vi "Post-Build Action.vi"(4 "measurement plugin service":refnum<class "Measurement Plugin Service.lvclass">, 5 "files generated by build":path[](array[path]), 6 "top level/always included VIs":path[](array[path]), 7 "destination path":path, 8 "error in":errorcluster, 9 "target name":string, 10 "build specification name":string, 11 "project path":path) -> (0 "error out":errorcluster)   [LabVIEW 2021, in "NI Measurement Plug-In SDK.lvlib"]
uses:
  NI Measurement Plug-In SDK.lvlib
  Measurement Plugin Service/Measurement Plugin Service.lvclass
  <vilib>/Utility/config.llb/Write Key (String).vi
  <vilib>/Utility/config.llb/NI_LVConfig.lvlib
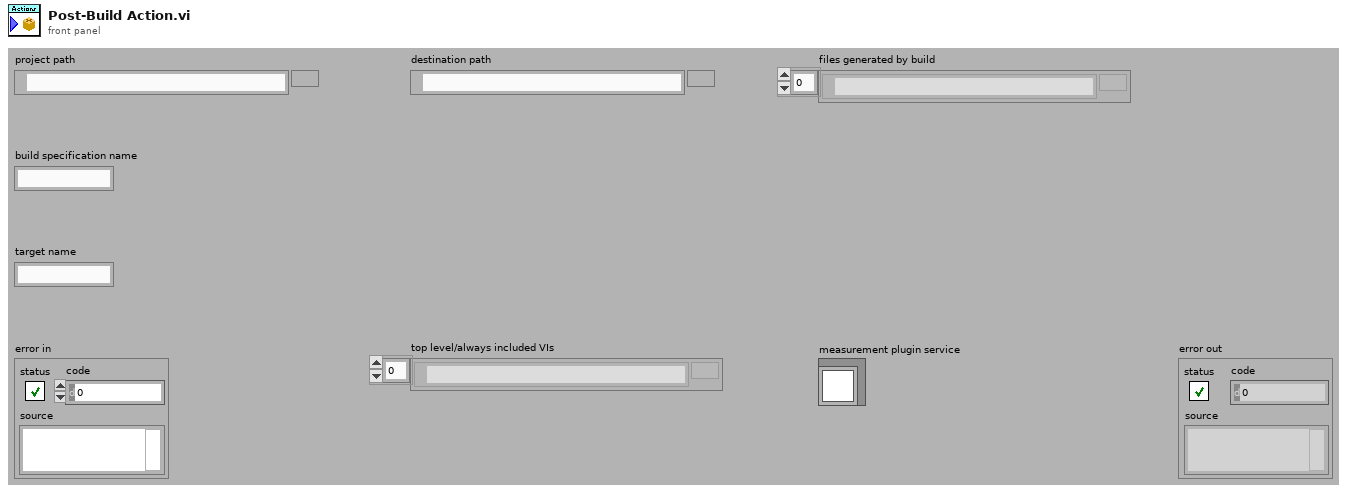
[diagram p1: front panel]
types:
  T1 = cluster{"target name":string, "top level/always included VIs":path[], "project path":path, "destination path":path, "build specification name":string, "files generated by build":path[]}
  T2 = typedef "NI Measurement Plug-In SDK.lvlib/User Interface Details.ctl" = cluster{"file url":string}
  T3 = typedef "NI Measurement Plug-In SDK.lvlib/Service Descriptor.ctl" = cluster{"measurement details":T4, "description URL":string, "service class":string, "measurement annotations":T5[]}
  T4 = typedef "NI Measurement Plug-In SDK.lvlib/Measurement Details.ctl" = cluster{"display name":string, "version":string}
  T5 = typedef "NI Measurement Plug-In SDK.lvlib/Measurement Annotation.ctl" = cluster{"key":string, "value":string}
  T6 = typedef "NI_LVConfig.lvlib/Config Data RefNum.ctl" = refnum<k1>
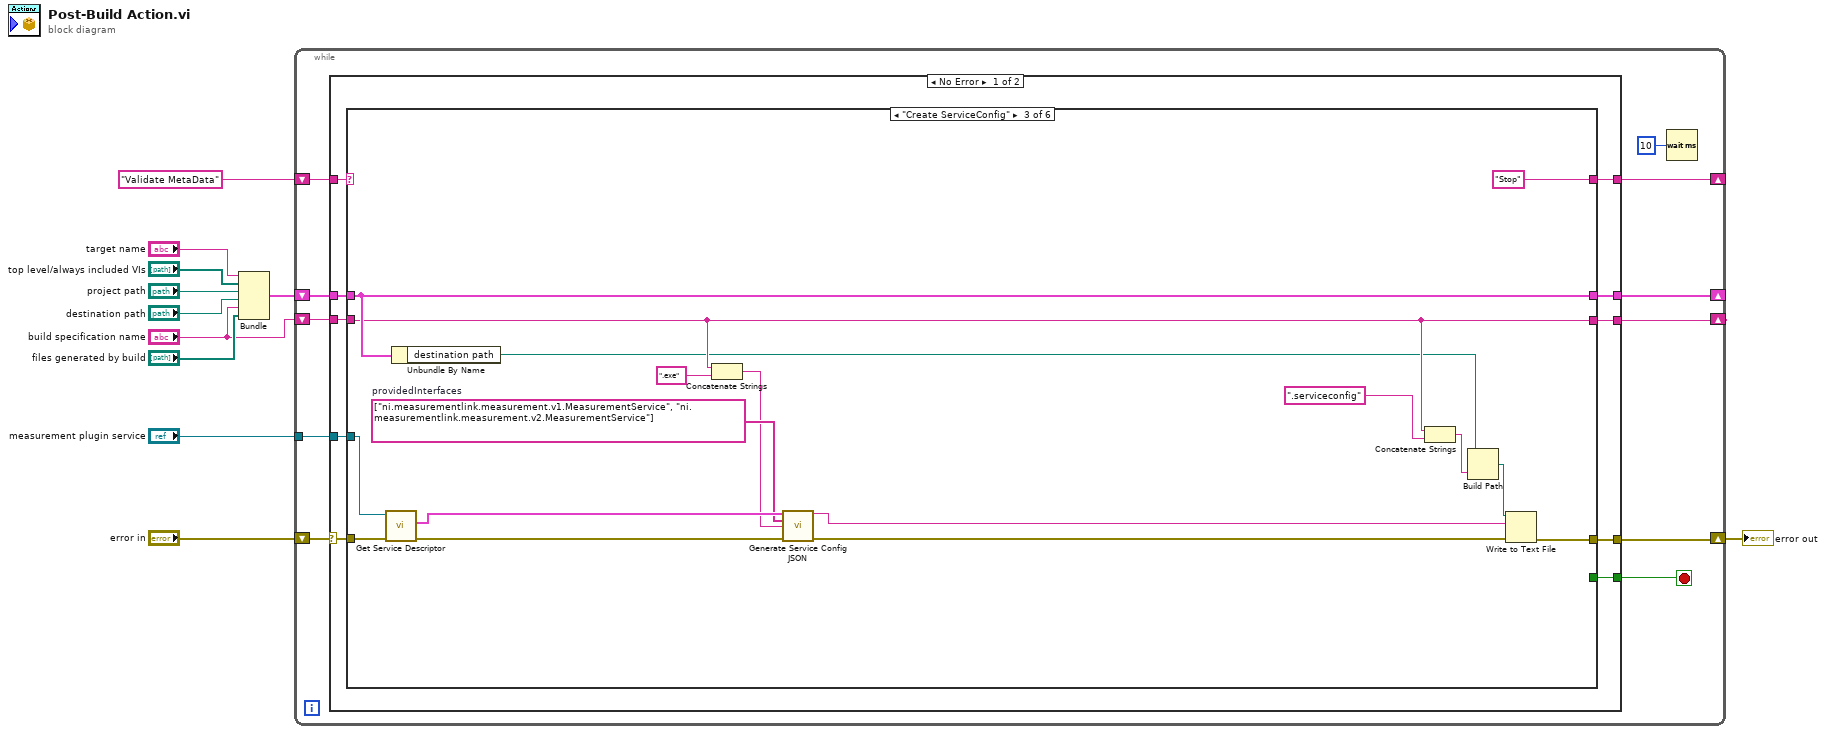
[diagram p0: block diagram]
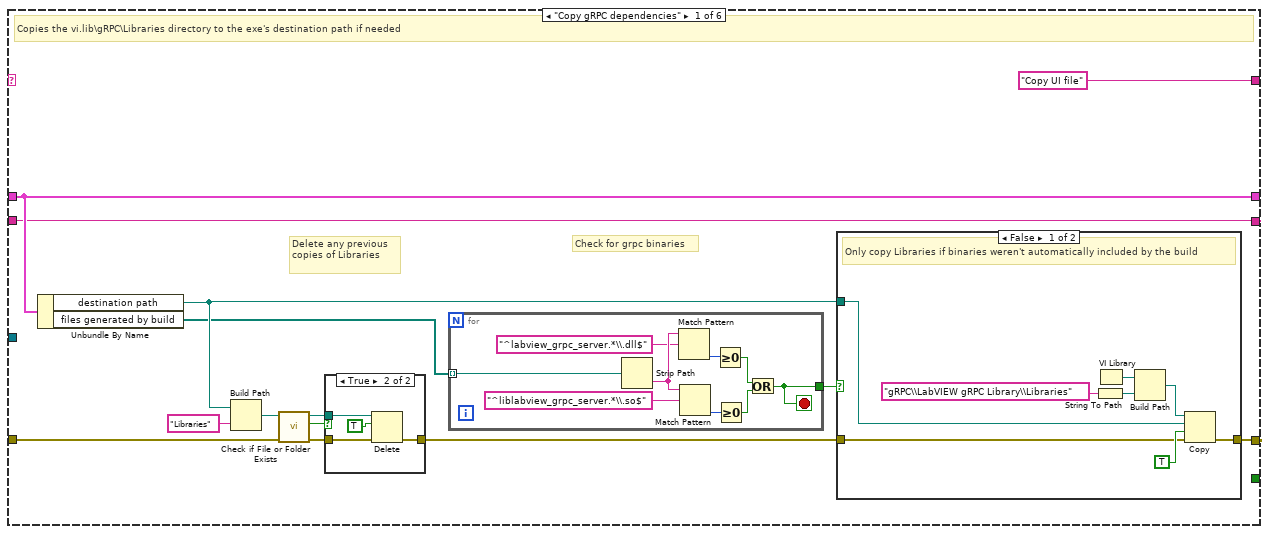
[diagram p2: hidden frame]
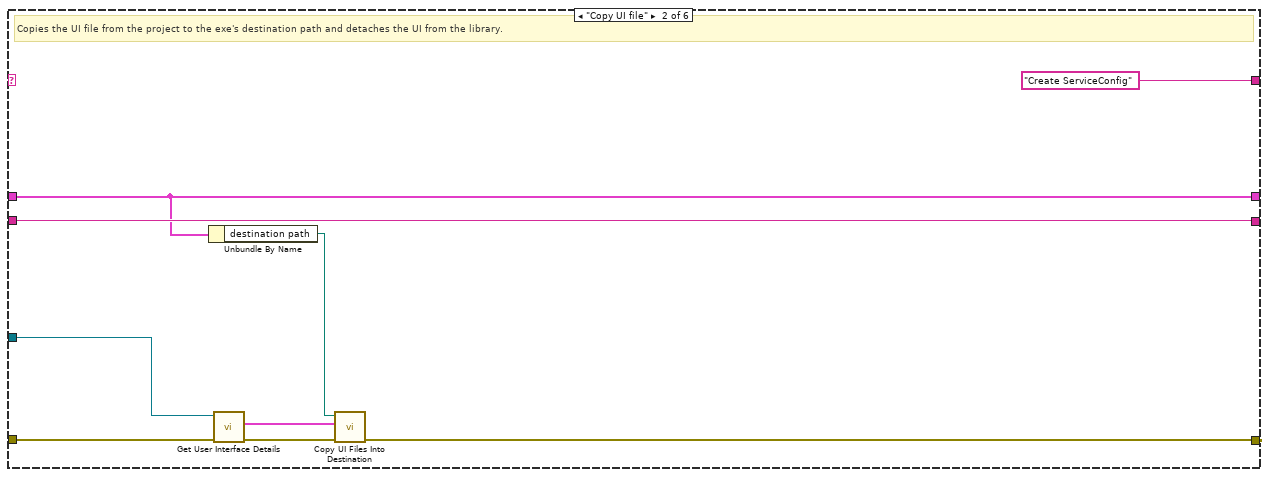
[diagram p5: hidden frame]
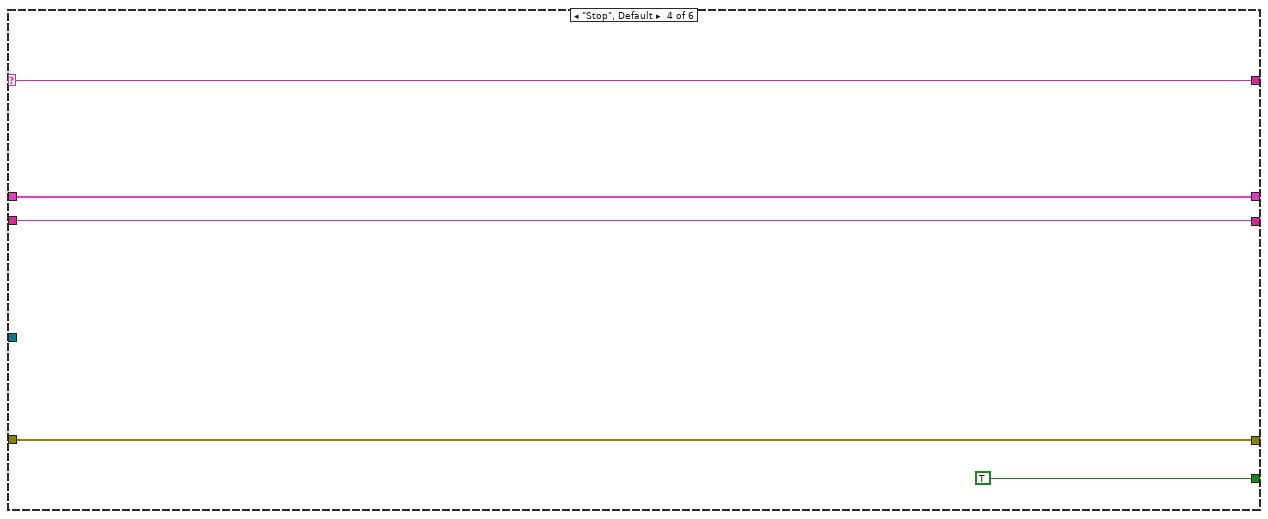
[diagram p6: hidden frame]
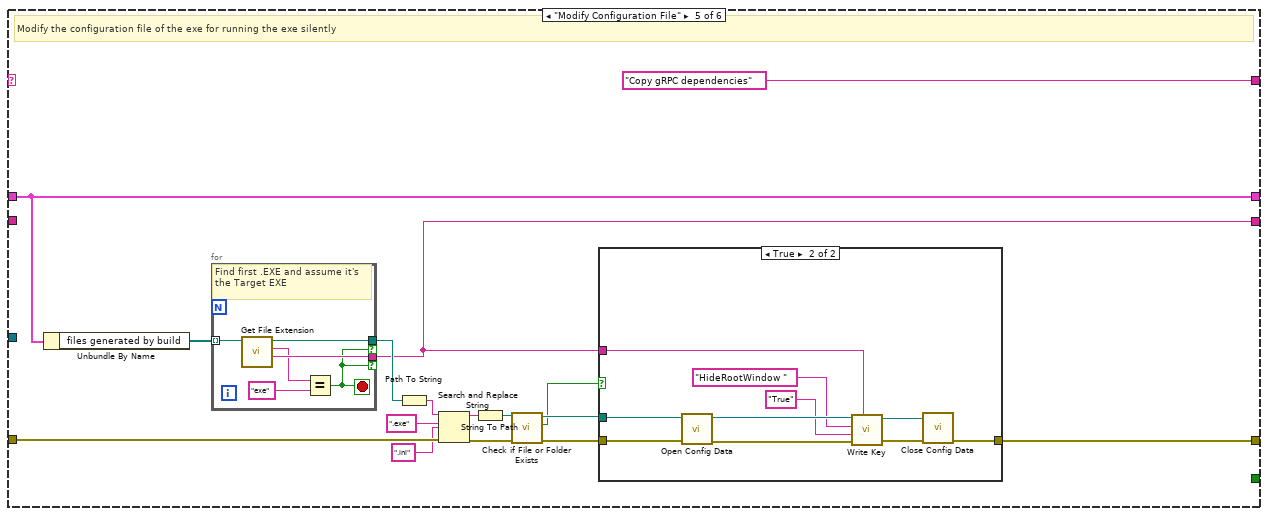
[diagram p7: hidden frame]
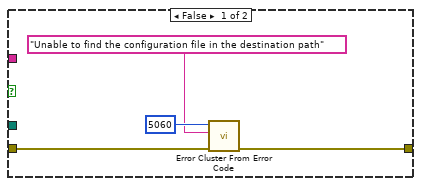
[diagram p8: hidden frame]
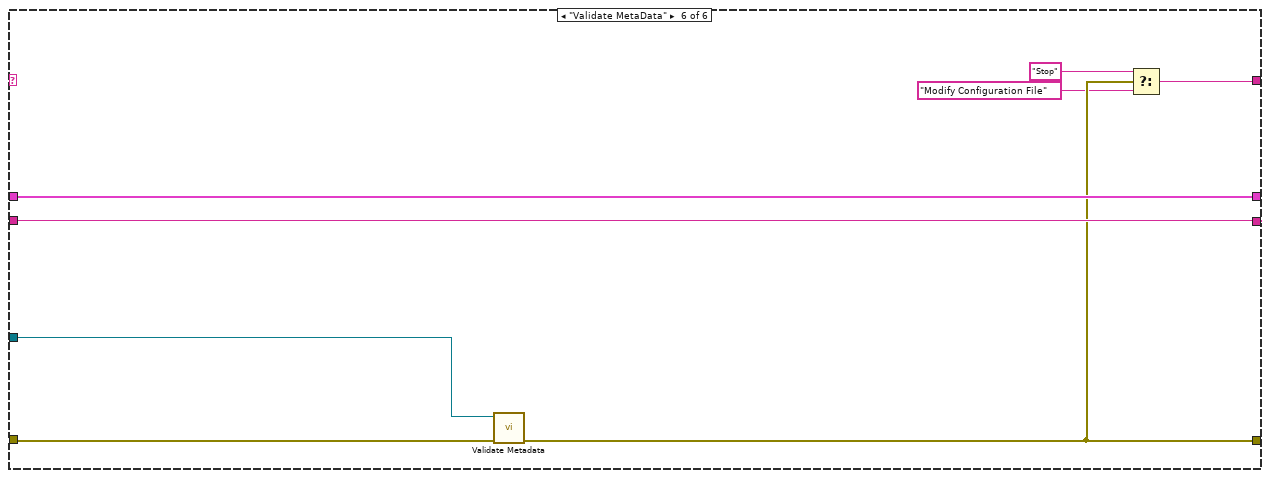
[diagram p9: hidden frame]
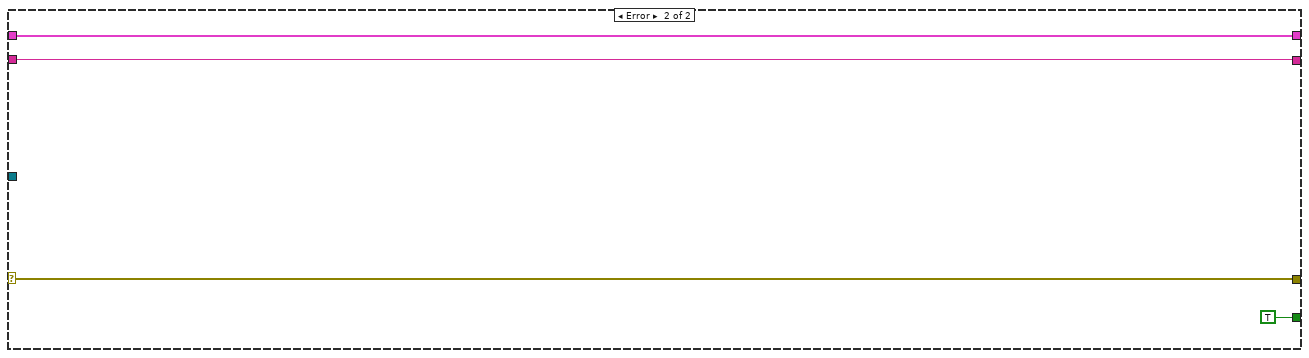
[diagram p10: hidden frame]
diagram:
  n1 = Bundle("target name"="target name", "top level/always included VIs"="top level/always included VIs", "project path"="project path", "destination path"="destination path", "build specification name"="build specification name", "files generated by build"="files generated by build") -> (w5:T1)  [unwired: 1 in]
  n2 = while {
    shift-right: [w19] -> _
    shift-left: w5 -> [w20]
    shift-right: [w18] -> w3
    shift-left: "error in" -> [w15]
    shift-right: [w17] -> _
    shift-left: "Validate MetaData" -> [w21]
    shift-right: [w14] -> _
    shift-left: "build specification name" -> [w13]
    tunnel: "measurement plugin service" -> [w12]
    stop <- w16 stop-if-true
    n3 = case shown="No Error" w15 {
      selector: w15 -> [w26 w147]
      tunnel: w21 -> [w32 _]
      tunnel: w20 -> [w31 w148]
      tunnel: [w30 w148] -> w19
      tunnel: [w29 w147] -> w18
      tunnel: [w28 _] -> w17
      tunnel: [w27 TRUE] -> w16
      tunnel: [w25 w145] -> w14
      tunnel: w13 -> [w24 w145]
      tunnel: w12 -> [w23 _]
      frame No Error {
        n4 = case shown="\"Create ServiceConfig\"" w32 {
          selector: w32 -> [_ _ _ w98 _ _]
          tunnel: w31 -> [w44 w75 w95 w100 w112 w144]
          tunnel: [w44 w75 w95 w100 w112 w144] -> w30
          tunnel: w26 -> [w36 w73 w85 w97 w110 w142]
          tunnel: [w46 w74 w88 w97 w116 w140] -> w29
          tunnel: ["Copy UI file" "Create ServiceConfig" "Stop" w98 "Copy gRPC dependencies" w137] -> w28
          tunnel: [_ _ _ TRUE _ _] -> w27
          tunnel: [w43 w77 w92 w96 w102 w143] -> w25
          tunnel: w24 -> [w43 w77 w92 w96 _ w143]
          tunnel: w23 -> [_ w71 w86 _ _ w141]
          frame "Copy gRPC dependencies" {
            # "Delete any previous copies of Libraries"
            # "Check for grpc binaries"
            # "Copies the vi.lib\\gRPC\\Libraries directory to the exe's destination path if needed"
            n5 = Unbundle By Name(w44) -> ("destination path"=w35:path, "files generated by build"=w33:path[])
            n6 = Build Path(base path=w35, name or relative path="Libraries") -> (appended path=w41:path)
            n7 = call <vilib>:"Check if File or Folder Exists.vi"("error in (no error)"=w36, "path"=w41) -> ("error out"=w40:errorcluster, "file or folder exists?"=w38:bool, "dup path"=w39:path)  [unwired: 7 in]
            n8 = case shown="True" w38 {
              tunnel: w40 -> [w56 w60]
              tunnel: [w56 w59] -> w34
              tunnel: w39 -> [_ w57]
              frame False {
              }
              frame True {
                n9 = Delete(path (use dialog)=w57, entire hierarchy (F)=TRUE ("confirm (F)"), error in=w60) -> (error out=w59:errorcluster)  [unwired: 2 in, 2 out]
              }
            }
            n10 = for {
              tunnel: [w47] -> w42
              tunnel: w33 -> [w52] mode=indexing
              stop <- w47 stop-if-true
              n11 = Strip Path(path=w52) -> (name=w55:string)  [unwired: 1 out]
              n12 = Match Pattern(string=w55, regular expression="^labview_grpc_server.*\\.dll$" ("pattern")) -> (offset past match=w51:i32)  [unwired: 1 in, 3 out]
              n13 = Match Pattern(string=w55, regular expression="^liblabview_grpc_server.*\\.so$" ("pattern")) -> (offset past match=w50:i32)  [unwired: 1 in, 3 out]
              n14 = Greater Or Equal To 0?(x=w51) -> (x >= 0?=w49:bool)
              n15 = Greater Or Equal To 0?(x=w50) -> (x >= 0?=w48:bool)
              n16 = Or(x=w49, y=w48) -> (x .or. y?=w47:bool)
            }
            n17 = case shown="False" w42 {
              tunnel: [w64 w69] -> w46
              tunnel: w35 -> [w62 _]
              tunnel: w34 -> [w61 w69]
              frame False {
                # "Only copy Libraries if binaries weren't automatically included by the build"
                n18 = String To Path(string="gRPC\\LabVIEW gRPC Library\\Libraries") -> (path=w66:path)
                n19 = VI Library() -> (path=w68:path)
                n20 = Build Path(base path=w68, name or relative path=w66) -> (appended path=w65:path)
                n21 = Copy(8:w61, 9:TRUE ("overwrite (F)"), 10:w62, 11:w65) -> (0:w64:errorcluster)  [unwired: 1 in, 2 out]
              }
              frame True {
              }
            }
          }
          frame "Copy UI file" {
            # "Copies the UI file from the project to the exe's destination path and detaches the UI from the library."
            n22 = Unbundle By Name(w75) -> ("destination path"=w76:path)
            n23 = call-dynamic "Get User Interface Details.vi"("error in"=w73, "measurement plugin service in"=w71) -> ("error out"=w72:errorcluster, "user interface details"=w70:T2[])  [unwired: 7 in, 1 out]
            n24 = call "Copy UI Files Into Destination.vi"("error in"=w72, "user interface details"=w70, "destination path"=w76) -> ("error out"=w74:errorcluster)  [unwired: 8 in]
          }
          frame "Create ServiceConfig" {
            w80 = string[] ["ni.measurementlink.measurement.v1.MeasurementService", "ni.measurementlink.measurement.v2.MeasurementService"]  # providedInterfaces
            n25 = call "Get Service Descriptor.vi"("error in"=w85, "measurement plugin service in"=w86) -> ("error out"=w84:errorcluster, "service descriptor"=w81:T3)  [unwired: 7 in, 1 out]
            n26 = Unbundle By Name(w95) -> ("destination path"=w90:path)
            n27 = Concatenate Strings(w92, ".exe" ("string")) -> (w79:string)
            n28 = call "Generate Service Config JSON.vi"("service descriptor"=w81, "provided interfaces"=w80, "path"=w79, "error in"=w84) -> ("service config JSON"=w82:string, "error out"=w83:errorcluster)  [unwired: 10 in]
            n29 = Concatenate Strings(w92, ".serviceconfig" ("string")) -> (w89:string)
            n30 = Build Path(base path=w90, name or relative path=w89) -> (appended path=w87:path)
            n31 = Write to Text File(file (use dialog)=w87, text=w82, error in=w83) -> (error out=w88:errorcluster)  [unwired: 1 in, 2 out]
          }
          frame "Stop", Default {
          }
          frame "Modify Configuration File" {
            # "Modify the configuration file of the exe for running the exe silently"
            n32 = Unbundle By Name(w112) -> ("files generated by build"=w111:path[])
            n33 = for {
              tunnel: w111 -> [w122] mode=indexing
              tunnel: [w121] -> w102 if=w117
              tunnel: [w120] -> w104 if=w117
              stop <- w117 stop-if-true
              # "Find first .EXE and assume it's the Target EXE"
              n34 = call <vilib>:"Get File Extension.vi"("file"=w122) -> ("filename without extension"=w121:string, "lowercase file extension"=w118:string, "dup file"=w120:path)  [unwired: 6 in, 2 out]
              n35 = Equal?(x=w118, y="exe") -> (x = y?=w117:bool)
            }
            n36 = Path To String(path=w104) -> (string=w103:string)
            n37 = Search and Replace String(input string=w103, search string=".exe", replace string=".ini", error in=w110) -> (result string=w107:string, error out=w109:errorcluster)  [unwired: 4 in, 2 out]
            n38 = String To Path(string=w107) -> (path=w106:path)
            n39 = call <vilib>:"Check if File or Folder Exists.vi"("error in (no error)"=w109, "path"=w106) -> ("error out"=w115:errorcluster, "file or folder exists?"=w113:bool, "dup path"=w114:path)  [unwired: 7 in]
            n40 = case shown="True" w113 {
              tunnel: [w125 w136] -> w116
              tunnel: w114 -> [_ w129]
              tunnel: w115 -> [w126 w128]
              tunnel: w102 -> [_ w127]
              frame False {
                n41 = call <vilib>:"Error Cluster From Error Code.vi"("error in (no error)"=w126, "error message (\"\")"="Unable to find the configuration file in the destination path" ("source"), "error code (0)"=5060) -> ("error out"=w125:errorcluster)  [unwired: 6 in]
              }
              frame True {
                n42 = call <vilib>:"Open Config Data.vi"("error in (no error)"=w128, "configuration file path"=w129) -> ("error out"=w135:errorcluster, "refnum"=w134:T6)  [unwired: 7 in, 1 out]
                n43 = call-poly <vilib>:"Write Key.vi"("section"=w127, "error in (no error)"=w135, "value"="True", "key"="HideRootWindow ", "refnum"=w134) -> ("error out"=w132:errorcluster, "refnum out"=w131:T6)  [unwired: 4 in, 1 out]
                n44 = call <vilib>:"Close Config Data.vi"("error in (no error)"=w132, "refnum"=w131) -> ("error out"=w136:errorcluster)  [unwired: 8 in, 1 out]
              }
            }
          }
          frame "Validate MetaData" {
            n45 = call "Validate Metadata.vi"("error in"=w142, "measurement plugin service in"=w141) -> ("error out"=w140:errorcluster)  [unwired: 8 in, 1 out]
            n46 = Select(t="Stop", s=w140, f="Modify Configuration File") -> (s? t:f=w137:string)
          }
        }
      }
      frame Error {
      }
    }
    n47 = Wait (ms)(milliseconds to wait=u32 10 ("millisecond timer value")) -> ()  [unwired: 1 out]
  }
  "error out" <- w3
